vi "Example TIF Read.vi"() -> ()   [LabVIEW 2016]
uses:
  ImageJ TIF Type Defs/TIF Read Image Information.ctl
panel:
  out "First Frame":u16[][](graph)
  in  "Read Type":enum32{"Read Frame", "Read Stack"}(radio)
  out "Image Info":T1
  out "Image Stack":u16[][][](array[numeric])
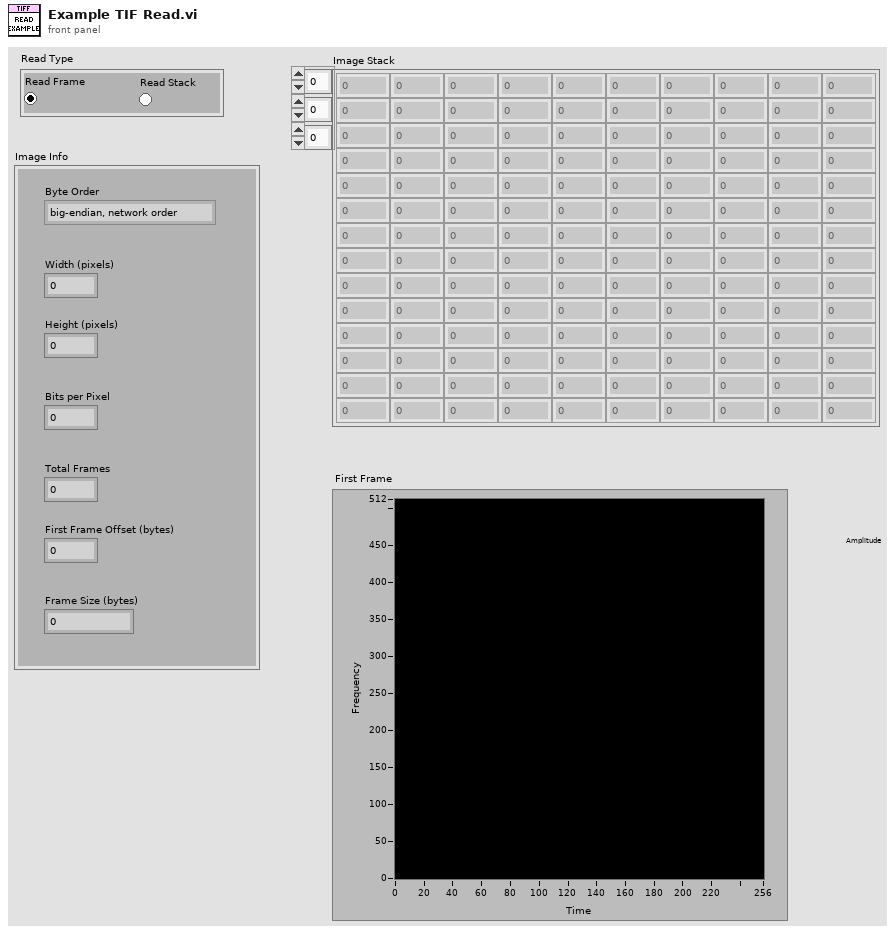
[diagram p1: front panel]
types:
  T1 = typedef "TIF Read Image Information.ctl" = cluster{"Byte Order":enum16{"big-endian, network order", "native, host order", "little-endian"}, "Width (pixels)":i32, "Height (pixels)":i32, "Bits per Pixel":u8, "Total Frames":u32, "First Frame Offset (bytes)":u32, "Frame Size (bytes)":u32}
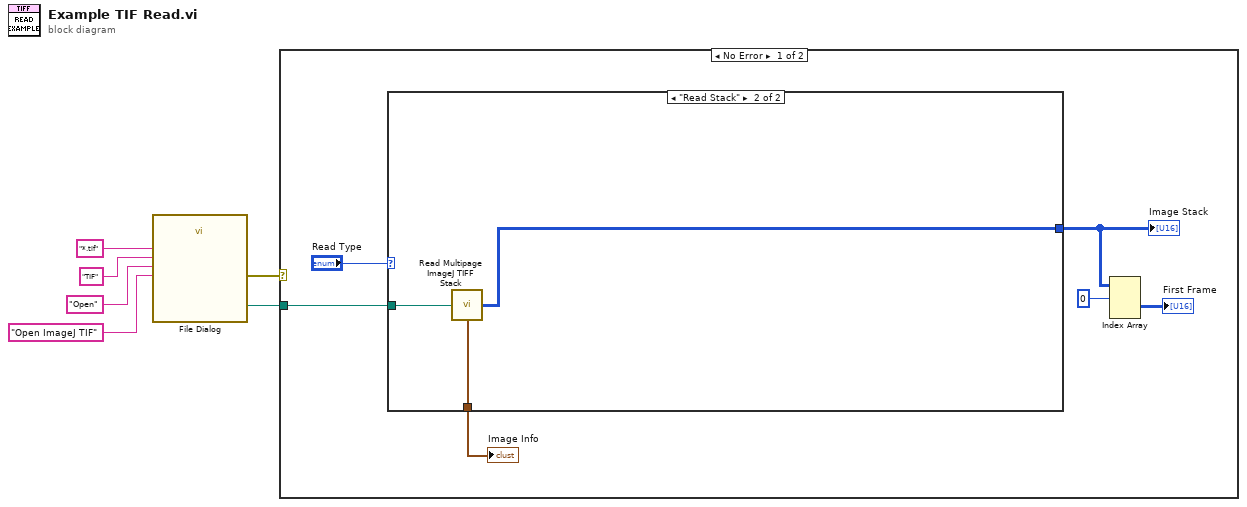
[diagram p0: block diagram]
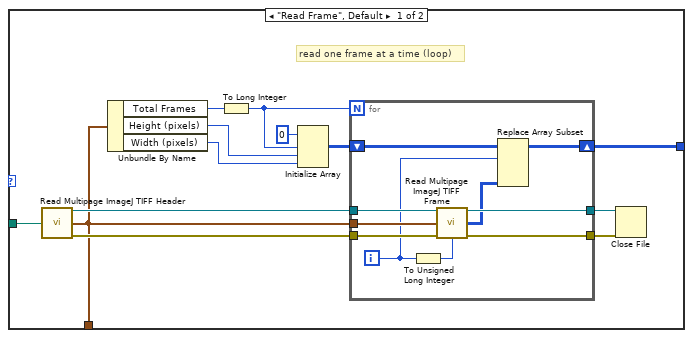
[diagram p2: hidden frame]
diagram:
  n1 = call "File Dialog"("prompt"="Open ImageJ TIF", "button label"="Open", "pattern (all files)"="*.tif", "pattern label"="TIF") -> ("selected path"=w1:path, "error out"=w2:errorcluster)  [unwired: 8 in, 2 out]
  n2 = case shown="No Error" w2 {
    tunnel: w1 -> [w12 _]
    frame No Error {
      n3 = case shown="\"Read Stack\"" "Read Type" {
        tunnel: w12 -> [w15 w38]
        tunnel: [w14 w37] -> w10
        tunnel: [w13 w36] -> w9
        frame "Read Frame", Default {
          # "read one frame at a time (loop)"
          n4 = call "Read Multipage ImageJ TIFF Header.vi"("TIFF Path"=w15) -> ("TIF Ref"=w21:refnum<file>, "Image Info"=w14:T1, "Error"=w22:errorcluster)  [unwired: 12 in]
          n5 = Unbundle By Name(w14) -> ("Total Frames"=w23:u32, "Height (pixels)"=w18:i32, "Width (pixels)"=w17:i32)
          n6 = To Long Integer(number=w23) -> (32bit integer=w16:i32)
          n7 = Initialize Array(u16 0 ("element"), w16, w18, w17) -> (w24:u16[][][])
          n8 = for {
            N: w16 -> [_]
            tunnel: w21 -> [w35]
            tunnel: w14 -> [w34]
            tunnel: w22 -> [w33]
            shift-right: [w28] -> w13
            shift-left: w24 -> [w29]
            tunnel: [w31] -> w25
            tunnel: [w30] -> w19
            i -> [w27]
            n9 = To Unsigned Long Integer(number=w27) -> (unsigned 32bit integer=w32:u32)
            n10 = call "Read Multipage ImageJ TIFF Frame.vi"("TIF Ref"=w35, "Image Info"=w34, "Error"=w33, "Frame"=w32) -> ("TIF Ref (Dup)"=w31:refnum<file>, "U16 Image"=w26:u16[][], "Error"=w30:errorcluster)  [unwired: 8 in, 1 out]
            n11 = Replace Array Subset(array=w29, new element=w26, index (dim 0)=w27) -> (w28:u16[][][])  [unwired: 2 in]
          }
          n12 = Close File(refnum=w25, error in=w19) -> ()  [unwired: 2 out]
        }
        frame "Read Stack" {
          n13 = call "Read Multipage ImageJ TIFF Stack.vi"("ImageJ Tif Path"=w38) -> ("U16 Stack"=w36:u16[][][], "Image Info"=w37:T1)  [unwired: 11 in, 2 out]
        }
      }
      "Image Info" <- w10
      "Image Stack" <- w9
      n14 = Index Array(array=w9, index (dim 0)=0 ("index (page)")) -> (element=→"First Frame":u16[][])  [unwired: 2 in]
    }
    frame Error {
    }
  }
